vi "Camera Messenger Regular.vi"(0 "Notifier Name":string, 1 "Binning":u16, 2 "General Camera Actions":T3, 5 "Exposure Time (s)":dbl, 7 "Save Path":path, 9 "No. of Frames":u32, 11 "Camera ROI":T1, 12 "Cooler On?":bool, 13 "Defect Correction On?":bool, 14 "Fan On?":bool) -> (3 "Current Exposure Time (s)":dbl, 4 "Notifier Name Dup":string, 6 "Running?":bool, 8 "Camera ROI":T1, 10 "Current Frame":u32, 15 "Image Ref":T2)   [LabVIEW 2016]
uses:
  Camera Controls/Generic Camera Actions.ctl
  Camera Controls/Generic Camera ROI.ctl
  <vilib>/vision/Image Controls.llb/IMAQ Image.ctl
  Hardware Configuration/Hardware Configuration Controls/Company.ctl
  Hamamatsu/Orca Flash/Orca Flash Controls/Orca Flash ROI.ctl
  Hamamatsu/Orca Flash/Orca Flash Controls/Orca Flash Parameters.ctl
  Hamamatsu/Orca Flash/Orca Flash Controls/Orca Flash Parameter List.ctl
  Hamamatsu/Orca Flash/Orca Flash Controls/Orca Flash Actions.ctl
  IDS/IDS Controls/IDS ROI.ctl
  IDS/IDS Controls/IDS Parameters.ctl
  IDS/IDS Controls/IDS Parameter List.ctl
  IDS/IDS Controls/IDS Actions.ctl
  Photometrics/Prime BSI/R Cubed SITK/Prime BSI R3 Controls/Prime R3 ROI.ctl
  Photometrics/Prime BSI/R Cubed SITK/Prime BSI R3 Controls/Prime R3 Parameters.ctl
  Photometrics/Prime BSI/R Cubed SITK/Prime BSI R3 Controls/Prime R3 Parameter List.ctl
  Photometrics/Prime BSI/R Cubed SITK/Prime BSI R3 Controls/Prime R3 Actions.ctl
  Camera Controls/Camera IMAQ Key Info.ctl
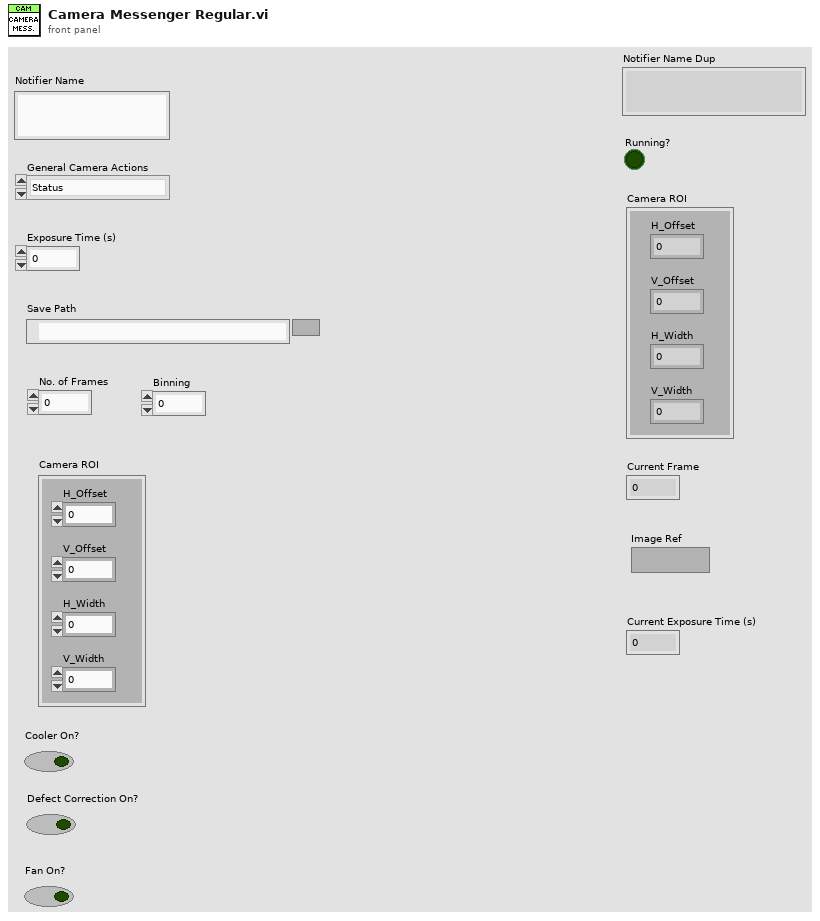
[diagram p1: front panel]
types:
  T1 = typedef "Generic Camera ROI.ctl" = cluster{"H_Offset":u16, "V_Offset":u16, "H_Width":u16, "V_Width":u16}
  T2 = typedef "IMAQ Image.ctl" = refnum<image>
  T3 = typedef "Generic Camera Actions.ctl" = enum16{"Status", "Live Preview", "Capture", "Abort", "Set Exposure Time (s)", "Get Exposure Time (s)", "Record Settings", "Binning", "Set ROI", "Get ROI", "Defect Correction On?", "Cooler On?", "Fan On?", "Quit"}
  T4 = typedef "Company.ctl" = enum16{"AA Opto Electronic", "ASI", "Coherent", "CVI", "DAQmx", "Hamamatsu", "IDS", "Mad City Labs", "Marzhauser", "Measurement Computing", "MPB Com", "Photometrics", "PI", "Prior", "Thorlabs"}
  T5 = typedef "Orca Flash Parameters.ctl" = cluster{"Value":dbl, "Parameter":T6}
  T6 = typedef "Orca Flash Parameter List.ctl" = u32
  T7 = typedef "Orca Flash ROI.ctl" = cluster{"H Offset":i32, "V Offset":i32, "H Width":i32, "V Width":i32}
  T8 = typedef "Orca Flash Actions.ctl" = enum16{"IDLE", "PREVIEW", "RECORD", "Record Settings", "SETPARAM", "GETPARAM", "SETROI", "GETROI", "PROGRESSIVE MODE", "AREA MODE", "STATUS", "QUIT"}
  T9 = typedef "IDS Parameter List.ctl" = enum16{"Exposure Time (s)", "Binning"}
  T10 = typedef "IDS Parameters.ctl" = cluster{"Parameter":T9, "Value":dbl}
  T11 = typedef "IDS ROI.ctl" = cluster{"H Offset":i32, "V Offset":i32, "H Width":i32, "V Width":i32}
  T12 = typedef "IDS Actions.ctl" = enum16{"Error Check", "Initialize", "Preview", "Record", "Abort", "Record Settings", "Set Parameter", "Get Parameter", "Set ROI", "Get ROI", "Status", "Quit"}
  T13 = typedef "Prime R3 Parameter List.ctl" = enum16{"Exposure Time (s)"}
  T14 = typedef "Prime R3 Parameters.ctl" = cluster{"Parameter":T13, "Value":dbl}
  T15 = typedef "Prime R3 ROI.ctl" = cluster{"X Start":u32, "X End":u32, "X Bin":u32, "Y Start":u32, "Y End":u32, "Y Bin":u32}
  T16 = typedef "Prime R3 Actions.ctl" = enum16{"Error Check", "Initialize", "Preview", "Record", "Abort", "Record Settings", "Set Parameter", "Get Parameter", "Set ROI", "Get ROI", "Status", "Set Trigger", "Quit"}
  T17 = typedef "Camera IMAQ Key Info.ctl" = cluster{"Frame":u32, "Sensor Height":i32, "Sensor Width":i32, "ROI Height":i32, "ROI Width":i32, "ROI Enable?":bool, "Bit per Pixel":u8}
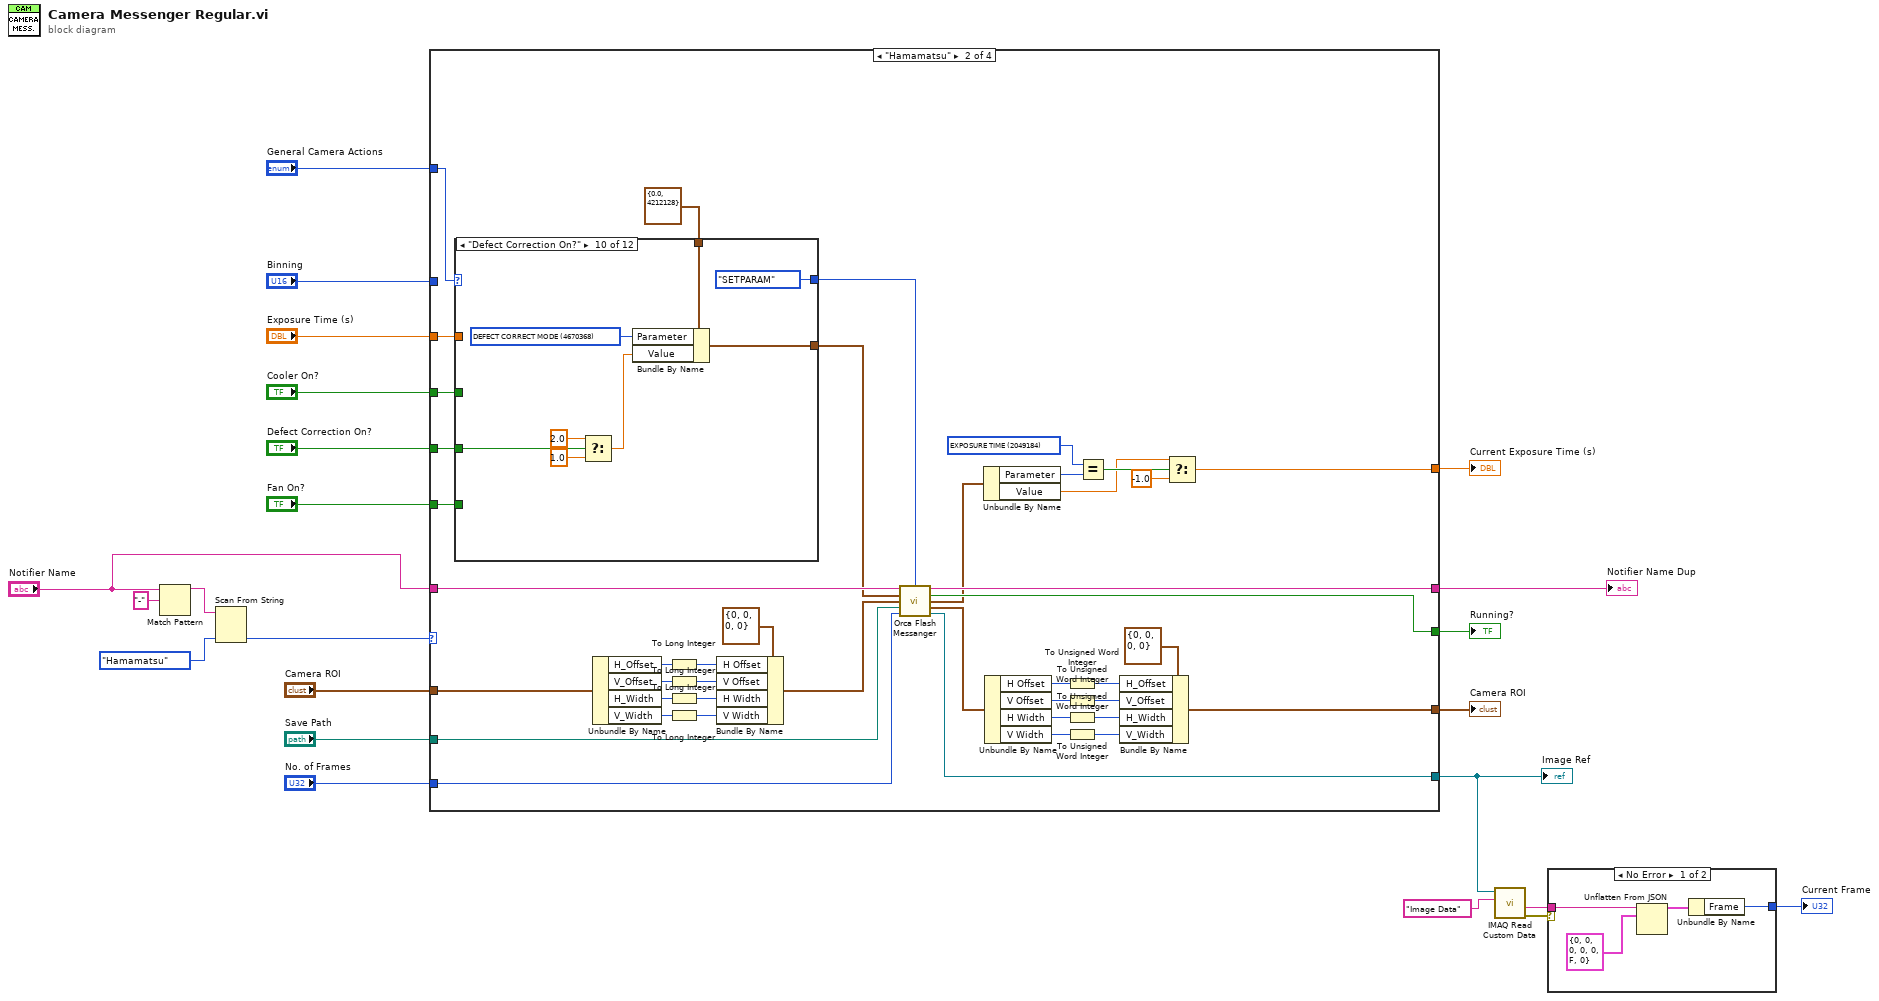
[diagram p0: block diagram]
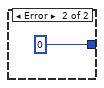
[diagram p2: hidden frame]
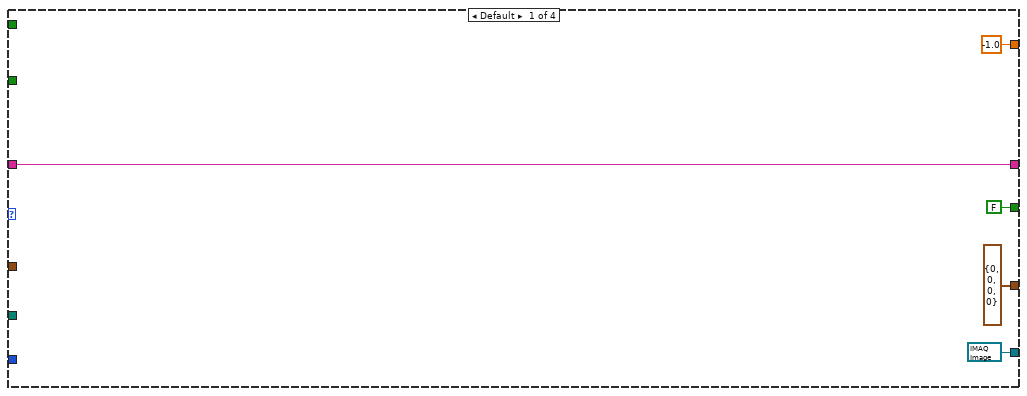
[diagram p3: hidden frame]
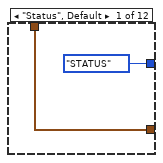
[diagram p4: hidden frame]
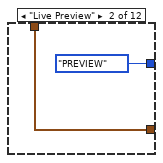
[diagram p5: hidden frame]
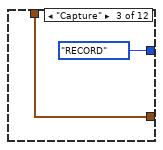
[diagram p6: hidden frame]
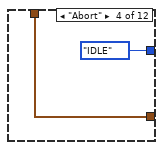
[diagram p7: hidden frame]
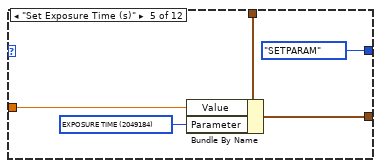
[diagram p8: hidden frame]
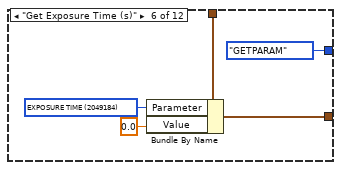
[diagram p9: hidden frame]
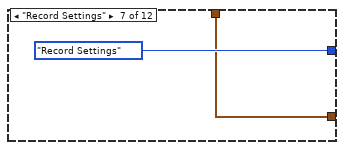
[diagram p10: hidden frame]
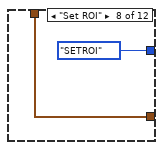
[diagram p11: hidden frame]
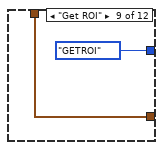
[diagram p12: hidden frame]
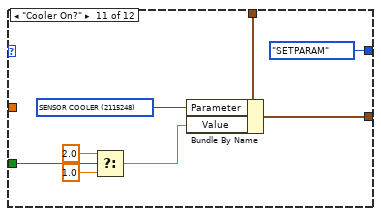
[diagram p13: hidden frame]
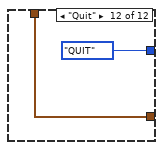
[diagram p14: hidden frame]
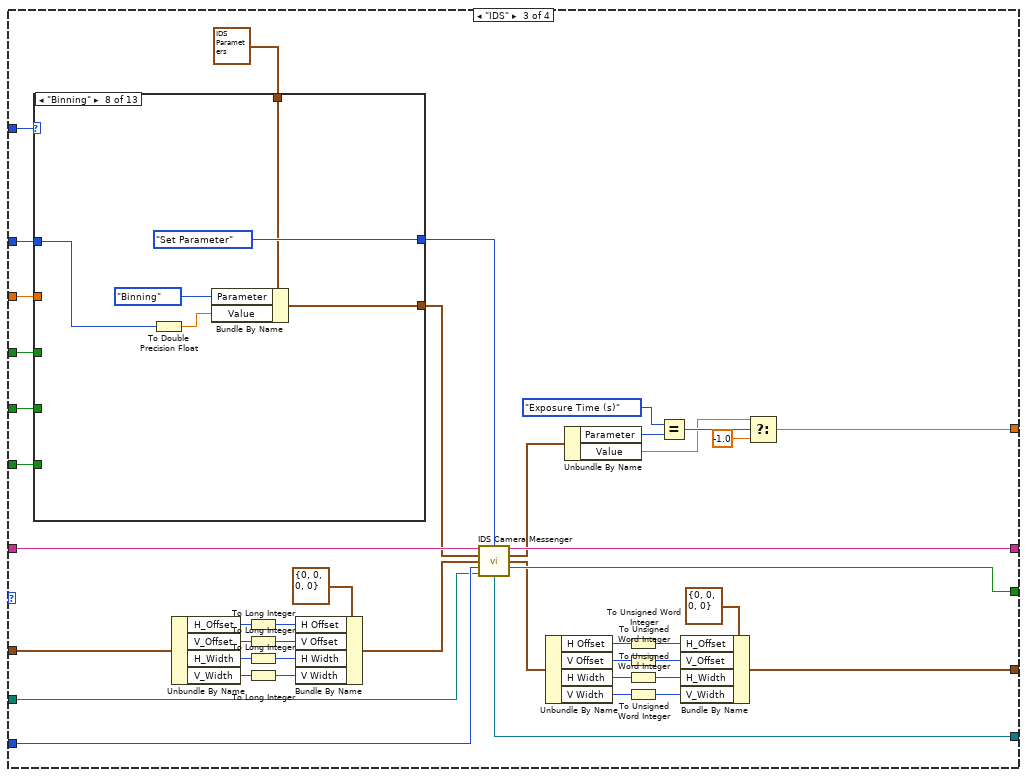
[diagram p15: hidden frame]
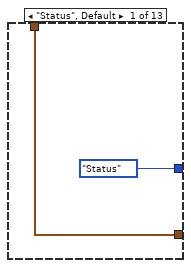
[diagram p16: hidden frame]
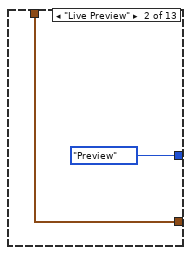
[diagram p17: hidden frame]
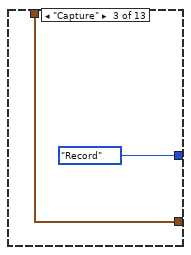
[diagram p18: hidden frame]
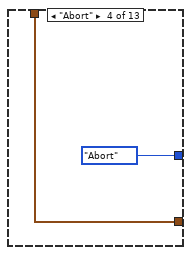
[diagram p19: hidden frame]
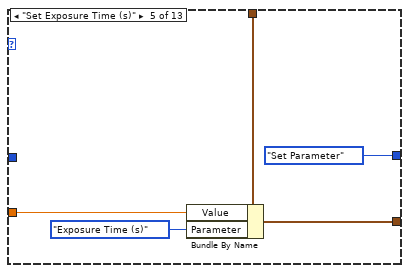
[diagram p20: hidden frame]
diagram:
  n1 = Match Pattern(string="Notifier Name", regular expression="-") -> (before substring=w20:string)  [unwired: 1 in, 3 out]
  n2 = Scan From String(input string=w20, default 1=Company."Hamamatsu" ("Company")) -> (output 1=w21:T4)  [unwired: 3 in, 3 out]
  n3 = case shown="\"Hamamatsu\"" w21 {
    tunnel: "Notifier Name" -> [w28 w71 w157 w239]
    tunnel: "General Camera Actions" -> [_ w56 w142 w232]
    tunnel: "No. of Frames" -> [_ w70 w156 w238]
    tunnel: "Save Path" -> [_ w69 w155 w210]
    tunnel: "Camera ROI" -> [_ w67 w153 w236]
    tunnel: [w28 w57 w143 w233] -> w15
    tunnel: "Exposure Time (s)" -> [_ w51 w138 w228]
    tunnel: "Cooler On?" -> [_ w55 w141 w231]
    tunnel: "Defect Correction On?" -> [_ w54 w140 w230]
    tunnel: "Fan On?" -> [_ w53 w139 w229]
    tunnel: [T2 refnum ("Image Ref") w48 w135 w225] -> w6
    tunnel: [FALSE ("Running?") w47 w134 w224] -> w10
    tunnel: [T1 {"H_Offset"=0, "V_Offset"=0, "H_Width"=0, "V_Width"=0} ("General Camera ROI") w36 w123 w213] -> w9
    tunnel: [-1.0 ("f") w30 w115 w195] -> w2
    tunnel: "Binning" -> [_ _ w114 _]
    frame Default {
    }
    frame "Hamamatsu" {
      w29 = T6 2049184 items=["SENSOR MODE"=4212128, "READOUT SPEED"=4211872, "READOUT DIRECTION"=4211904, "TRIGGER GLOBAL EXPOSURE"=2049680, "TRIGGER DELAY"=1066480, "SYNC READOUT SYSTEM BLANK"=1066528, "SENSOR COOLER"=2115248, "SENSOR COOLER STATUS"=2115280, "EXPOSURE TIME"=2049184, "DEFECT CORRECT MODE"=4670368, "BINNING"=4215968, "INTERNAL LINE SPEED"=4226000, "INTERNAL LINE INTERVAL"=4226016, "IMAGE PIXEL TYPE"=4343296, "NUMBER OF OUTPUT TRIGGER CONNECTOR"=1852320, "OUTPUT TRIGGER SOURCE[0]"=1852576, "OUTPUT TRIGGER SOURCE[1]"=1852832, "OUTPUT TRIGGER SOURCE[2]"=1853088, "OUTPUT TRIGGER POLARITY[0]"=1852592, "OUTPUT TRIGGER POLARITY[1]"=1852848, "OUTPUT TRIGGER POLARITY[2]"=1853104, "OUTPUT TRIGGER ACTIVE[0]"=1852608, "OUTPUT TRIGGER ACTIVE[1]"=1852864, "OUTPUT TRIGGER ACTIVE[2]"=1853120, "OUTPUT TRIGGER DELAY[0]"=1852624, "OUTPUT TRIGGER DELAY[1]"=1852880, "OUTPUT TRIGGER DELAY[2]"=1853136, "OUTPUT TRIGGER PERIOD[0]"=1852640, "OUTPUT TRIGGER PERIOD[1]"=1852896, "OUTPUT TRIGGER PERIOD[2]"=1853152, "OUTPUT TRIGGER KIND[0]"=1852656, "OUTPUT TRIGGER KIND[1]"=1852912, "OUTPUT TRIGGER KIND[2]"=1853168, "OUTPUT TRIGGER PRE HSYNC COUNT"=1852704] ("x")
      n4 = case shown="\"Defect Correction On?\"" w56 {
        tunnel: w55 -> [_ _ _ _ _ _ _ _ _ _ w108 _]
        tunnel: w54 -> [_ _ _ _ _ _ _ _ _ w99 _ _]
        tunnel: w53 -> [_ _ _ _ _ _ _ _ _ _ _ _]
        tunnel: [Orca_Flash_Actions."STATUS" ("Camera Actions") Orca_Flash_Actions."PREVIEW" ("Camera Actions") Orca_Flash_Actions."RECORD" ("Camera Actions") Orca_Flash_Actions."IDLE" ("Camera Actions") Orca_Flash_Actions."SETPARAM" ("Camera Actions") Orca_Flash_Actions."GETPARAM" ("Camera Actions") Orca_Flash_Actions."Record Settings" ("Camera Actions") Orca_Flash_Actions."SETROI" ("Camera Actions") Orca_Flash_Actions."GETROI" ("Camera Actions") Orca_Flash_Actions."SETPARAM" ("Camera Actions") Orca_Flash_Actions."SETPARAM" ("Camera Actions") Orca_Flash_Actions."QUIT" ("Camera Actions")] -> w52
        tunnel: w51 -> [_ _ _ _ w83 _ _ _ _ _ _ _]
        tunnel: [w72 w74 w76 w78 w82 w88 w90 w92 w94 w101 w104 w113] -> w50
        tunnel: T5 {"Value"=0.0, "Parameter"=4212128} ("sCMOS Parameter") -> [w72 w74 w76 w78 w81 w89 w90 w92 w94 w102 w110 w113]
        frame "Status", Default {
        }
        frame "Live Preview" {
        }
        frame "Capture" {
        }
        frame "Abort" {
        }
        frame "Set Exposure Time (s)" {
          w80 = T6 2049184 items=["SENSOR MODE"=4212128, "READOUT SPEED"=4211872, "READOUT DIRECTION"=4211904, "TRIGGER GLOBAL EXPOSURE"=2049680, "TRIGGER DELAY"=1066480, "SYNC READOUT SYSTEM BLANK"=1066528, "SENSOR COOLER"=2115248, "SENSOR COOLER STATUS"=2115280, "EXPOSURE TIME"=2049184, "DEFECT CORRECT MODE"=4670368, "BINNING"=4215968, "INTERNAL LINE SPEED"=4226000, "INTERNAL LINE INTERVAL"=4226016, "IMAGE PIXEL TYPE"=4343296, "NUMBER OF OUTPUT TRIGGER CONNECTOR"=1852320, "OUTPUT TRIGGER SOURCE[0]"=1852576, "OUTPUT TRIGGER SOURCE[1]"=1852832, "OUTPUT TRIGGER SOURCE[2]"=1853088, "OUTPUT TRIGGER POLARITY[0]"=1852592, "OUTPUT TRIGGER POLARITY[1]"=1852848, "OUTPUT TRIGGER POLARITY[2]"=1853104, "OUTPUT TRIGGER ACTIVE[0]"=1852608, "OUTPUT TRIGGER ACTIVE[1]"=1852864, "OUTPUT TRIGGER ACTIVE[2]"=1853120, "OUTPUT TRIGGER DELAY[0]"=1852624, "OUTPUT TRIGGER DELAY[1]"=1852880, "OUTPUT TRIGGER DELAY[2]"=1853136, "OUTPUT TRIGGER PERIOD[0]"=1852640, "OUTPUT TRIGGER PERIOD[1]"=1852896, "OUTPUT TRIGGER PERIOD[2]"=1853152, "OUTPUT TRIGGER KIND[0]"=1852656, "OUTPUT TRIGGER KIND[1]"=1852912, "OUTPUT TRIGGER KIND[2]"=1853168, "OUTPUT TRIGGER PRE HSYNC COUNT"=1852704] ("Parameter")
          n5 = Bundle By Name(cluster=w81, "Value"=w83, "Parameter"=w80) -> (w82:T5)
        }
        frame "Get Exposure Time (s)" {
          w86 = T6 2049184 items=["SENSOR MODE"=4212128, "READOUT SPEED"=4211872, "READOUT DIRECTION"=4211904, "TRIGGER GLOBAL EXPOSURE"=2049680, "TRIGGER DELAY"=1066480, "SYNC READOUT SYSTEM BLANK"=1066528, "SENSOR COOLER"=2115248, "SENSOR COOLER STATUS"=2115280, "EXPOSURE TIME"=2049184, "DEFECT CORRECT MODE"=4670368, "BINNING"=4215968, "INTERNAL LINE SPEED"=4226000, "INTERNAL LINE INTERVAL"=4226016, "IMAGE PIXEL TYPE"=4343296, "NUMBER OF OUTPUT TRIGGER CONNECTOR"=1852320, "OUTPUT TRIGGER SOURCE[0]"=1852576, "OUTPUT TRIGGER SOURCE[1]"=1852832, "OUTPUT TRIGGER SOURCE[2]"=1853088, "OUTPUT TRIGGER POLARITY[0]"=1852592, "OUTPUT TRIGGER POLARITY[1]"=1852848, "OUTPUT TRIGGER POLARITY[2]"=1853104, "OUTPUT TRIGGER ACTIVE[0]"=1852608, "OUTPUT TRIGGER ACTIVE[1]"=1852864, "OUTPUT TRIGGER ACTIVE[2]"=1853120, "OUTPUT TRIGGER DELAY[0]"=1852624, "OUTPUT TRIGGER DELAY[1]"=1852880, "OUTPUT TRIGGER DELAY[2]"=1853136, "OUTPUT TRIGGER PERIOD[0]"=1852640, "OUTPUT TRIGGER PERIOD[1]"=1852896, "OUTPUT TRIGGER PERIOD[2]"=1853152, "OUTPUT TRIGGER KIND[0]"=1852656, "OUTPUT TRIGGER KIND[1]"=1852912, "OUTPUT TRIGGER KIND[2]"=1853168, "OUTPUT TRIGGER PRE HSYNC COUNT"=1852704] ("Parameter")
          n6 = Bundle By Name(cluster=w89, "Parameter"=w86, "Value"=0.0) -> (w88:T5)
        }
        frame "Record Settings" {
        }
        frame "Set ROI" {
        }
        frame "Get ROI" {
        }
        frame "Defect Correction On?" {
          w100 = T6 4670368 items=["SENSOR MODE"=4212128, "READOUT SPEED"=4211872, "READOUT DIRECTION"=4211904, "TRIGGER GLOBAL EXPOSURE"=2049680, "TRIGGER DELAY"=1066480, "SYNC READOUT SYSTEM BLANK"=1066528, "SENSOR COOLER"=2115248, "SENSOR COOLER STATUS"=2115280, "EXPOSURE TIME"=2049184, "DEFECT CORRECT MODE"=4670368, "BINNING"=4215968, "INTERNAL LINE SPEED"=4226000, "INTERNAL LINE INTERVAL"=4226016, "IMAGE PIXEL TYPE"=4343296, "NUMBER OF OUTPUT TRIGGER CONNECTOR"=1852320, "OUTPUT TRIGGER SOURCE[0]"=1852576, "OUTPUT TRIGGER SOURCE[1]"=1852832, "OUTPUT TRIGGER SOURCE[2]"=1853088, "OUTPUT TRIGGER POLARITY[0]"=1852592, "OUTPUT TRIGGER POLARITY[1]"=1852848, "OUTPUT TRIGGER POLARITY[2]"=1853104, "OUTPUT TRIGGER ACTIVE[0]"=1852608, "OUTPUT TRIGGER ACTIVE[1]"=1852864, "OUTPUT TRIGGER ACTIVE[2]"=1853120, "OUTPUT TRIGGER DELAY[0]"=1852624, "OUTPUT TRIGGER DELAY[1]"=1852880, "OUTPUT TRIGGER DELAY[2]"=1853136, "OUTPUT TRIGGER PERIOD[0]"=1852640, "OUTPUT TRIGGER PERIOD[1]"=1852896, "OUTPUT TRIGGER PERIOD[2]"=1853152, "OUTPUT TRIGGER KIND[0]"=1852656, "OUTPUT TRIGGER KIND[1]"=1852912, "OUTPUT TRIGGER KIND[2]"=1853168, "OUTPUT TRIGGER PRE HSYNC COUNT"=1852704] ("Parameter")
          n7 = Select(t=2.0, s=w99, f=1.0) -> (s? t:f=w96:dbl)
          n8 = Bundle By Name(cluster=w102, "Parameter"=w100, "Value"=w96) -> (w101:T5)
        }
        frame "Cooler On?" {
          w109 = T6 2115248 items=["SENSOR MODE"=4212128, "READOUT SPEED"=4211872, "READOUT DIRECTION"=4211904, "TRIGGER GLOBAL EXPOSURE"=2049680, "TRIGGER DELAY"=1066480, "SYNC READOUT SYSTEM BLANK"=1066528, "SENSOR COOLER"=2115248, "SENSOR COOLER STATUS"=2115280, "EXPOSURE TIME"=2049184, "DEFECT CORRECT MODE"=4670368, "BINNING"=4215968, "INTERNAL LINE SPEED"=4226000, "INTERNAL LINE INTERVAL"=4226016, "IMAGE PIXEL TYPE"=4343296, "NUMBER OF OUTPUT TRIGGER CONNECTOR"=1852320, "OUTPUT TRIGGER SOURCE[0]"=1852576, "OUTPUT TRIGGER SOURCE[1]"=1852832, "OUTPUT TRIGGER SOURCE[2]"=1853088, "OUTPUT TRIGGER POLARITY[0]"=1852592, "OUTPUT TRIGGER POLARITY[1]"=1852848, "OUTPUT TRIGGER POLARITY[2]"=1853104, "OUTPUT TRIGGER ACTIVE[0]"=1852608, "OUTPUT TRIGGER ACTIVE[1]"=1852864, "OUTPUT TRIGGER ACTIVE[2]"=1853120, "OUTPUT TRIGGER DELAY[0]"=1852624, "OUTPUT TRIGGER DELAY[1]"=1852880, "OUTPUT TRIGGER DELAY[2]"=1853136, "OUTPUT TRIGGER PERIOD[0]"=1852640, "OUTPUT TRIGGER PERIOD[1]"=1852896, "OUTPUT TRIGGER PERIOD[2]"=1853152, "OUTPUT TRIGGER KIND[0]"=1852656, "OUTPUT TRIGGER KIND[1]"=1852912, "OUTPUT TRIGGER KIND[2]"=1853168, "OUTPUT TRIGGER PRE HSYNC COUNT"=1852704] ("Parameter")
          n9 = Select(t=2.0, s=w108, f=1.0) -> (s? t:f=w105:dbl)
          n10 = Bundle By Name(cluster=w110, "Parameter"=w109, "Value"=w105) -> (w104:T5)
        }
        frame "Quit" {
        }
      }
      n11 = Unbundle By Name(w67) -> ("H_Offset"=w63:u16, "V_Offset"=w64:u16, "H_Width"=w65:u16, "V_Width"=w66:u16)
      n12 = To Long Integer(number=w63) -> (32bit integer=w62:i32)
      n13 = To Long Integer(number=w64) -> (32bit integer=w61:i32)
      n14 = To Long Integer(number=w65) -> (32bit integer=w60:i32)
      n15 = To Long Integer(number=w66) -> (32bit integer=w59:i32)
      n16 = Bundle By Name(cluster=T7 {"H Offset"=0, "V Offset"=0, "H Width"=0, "V Width"=0} ("sCMOS ROI"), "H Offset"=w62, "V Offset"=w61, "H Width"=w60, "V Width"=w59) -> (w58:T7)
      n17 = call "Orca Flash Messanger.vi"("Notifier Name"=w71, "Camera Actions"=w52, "sCMOS Parameter"=w50, "sCMOS ROI"=w58, "Path"=w69, "# of frames"=w70) -> ("Notifier Name Dup"=w57:string, "Running?"=w47:bool, "sCMOS Parameter"=w31:T5, "sCMOS ROI"=w45:T7, "Image Ref"=w48:T2)  [unwired: 5 in]
      n18 = Unbundle By Name(w31) -> ("Parameter"=w35:T6, "Value"=w33:dbl)
      n19 = Unbundle By Name(w45) -> ("H Offset"=w44:i32, "V Offset"=w43:i32, "H Width"=w42:i32, "V Width"=w41:i32)
      n20 = To Unsigned Word Integer(number=w44) -> (unsigned 16bit integer=w40:u16)
      n21 = To Unsigned Word Integer(number=w43) -> (unsigned 16bit integer=w39:u16)
      n22 = To Unsigned Word Integer(number=w42) -> (unsigned 16bit integer=w38:u16)
      n23 = To Unsigned Word Integer(number=w41) -> (unsigned 16bit integer=w37:u16)
      n24 = Equal?(x=w29, y=w35) -> (x = y?=w34:bool)
      n25 = Bundle By Name(cluster=T1 {"H_Offset"=0, "V_Offset"=0, "H_Width"=0, "V_Width"=0} ("General Camera ROI"), "H_Offset"=w40, "V_Offset"=w39, "H_Width"=w38, "V_Width"=w37) -> (w36:T1)
      n26 = Select(t=w33, s=w34, f=-1.0) -> (s? t:f=w30:dbl)
    }
    frame "IDS" {
      n27 = case shown="\"Binning\"" w142 {
        tunnel: w141 -> [_ _ _ _ _ _ _ _ _ _ _ _ _]
        tunnel: w140 -> [_ _ _ _ _ _ _ _ _ _ _ _ _]
        tunnel: w139 -> [_ _ _ _ _ _ _ _ _ _ _ _ _]
        tunnel: [IDS_Actions."Status" ("IDS Actions") IDS_Actions."Preview" ("IDS Actions") IDS_Actions."Record" ("IDS Actions") IDS_Actions."Abort" ("IDS Actions") IDS_Actions."Set Parameter" ("IDS Actions") IDS_Actions."Get Parameter" ("IDS Actions") IDS_Actions."Record Settings" ("IDS Actions") IDS_Actions."Set Parameter" ("IDS Actions") IDS_Actions."Set ROI" ("IDS Actions") IDS_Actions."Get ROI" ("IDS Actions") IDS_Actions."Status" ("IDS Actions") IDS_Actions."Status" ("IDS Actions") IDS_Actions."Quit" ("IDS Actions")] -> w122
        tunnel: w138 -> [_ _ _ _ w170 _ _ _ _ _ _ _ _]
        tunnel: [w159 w161 w163 w165 w169 w171 w177 w181 w185 w187 w189 w191 w193] -> w137
        tunnel: T10 {"Parameter"=enum."Exposure Time (s)", "Value"=4212128.0} ("IDS Parameter") -> [w159 w161 w163 w165 w168 w174 w177 w182 w185 w187 w189 w191 w193]
        tunnel: w114 -> [_ _ _ _ _ _ _ w178 _ _ _ _ _]
        frame "Status", Default {
        }
        frame "Live Preview" {
        }
        frame "Capture" {
        }
        frame "Abort" {
        }
        frame "Set Exposure Time (s)" {
          n28 = Bundle By Name(cluster=w168, "Value"=w170, "Parameter"=IDS_Parameter_List."Exposure Time (s)") -> (w169:T10)
        }
        frame "Get Exposure Time (s)" {
          n29 = Bundle By Name(cluster=w174, "Parameter"=IDS_Parameter_List."Exposure Time (s)", "Value"=0.0) -> (w171:T10)
        }
        frame "Record Settings" {
        }
        frame "Binning" {
          n30 = To Double Precision Float(number=w178) -> (double precision float=w179:dbl)
          n31 = Bundle By Name(cluster=w182, "Parameter"=IDS_Parameter_List."Binning", "Value"=w179) -> (w181:T10)
        }
        frame "Set ROI" {
        }
        frame "Get ROI" {
        }
        frame "Defect Correction On?" {
        }
        frame "Cooler On?" {
        }
        frame "Quit" {
        }
      }
      n32 = Unbundle By Name(w153) -> ("H_Offset"=w149:u16, "V_Offset"=w150:u16, "H_Width"=w151:u16, "V_Width"=w152:u16)
      n33 = To Long Integer(number=w149) -> (32bit integer=w148:i32)
      n34 = To Long Integer(number=w150) -> (32bit integer=w147:i32)
      n35 = To Long Integer(number=w151) -> (32bit integer=w146:i32)
      n36 = To Long Integer(number=w152) -> (32bit integer=w145:i32)
      n37 = Bundle By Name(cluster=T11 {"H Offset"=0, "V Offset"=0, "H Width"=0, "V Width"=0} ("sCMOS ROI"), "H Offset"=w148, "V Offset"=w147, "H Width"=w146, "V Width"=w145) -> (w144:T11)
      n38 = call "IDS Camera Messenger.vi"("Notifier Name"=w157, "IDS Actions"=w122, "IDS Parameter"=w137, "ROI Setup"=w144, "# of Frames"=w156, "File Save Path"=w155) -> ("Notifier Name (Dup)"=w143:string, "IDS Parameter"=w121:T10, "IDS ROI"=w132:T11, "Running?"=w134:bool, "Image Ref"=w135:T2)  [unwired: 4 in, 1 out]
      n39 = Unbundle By Name(w132) -> ("H Offset"=w131:i32, "V Offset"=w130:i32, "H Width"=w129:i32, "V Width"=w128:i32)
      n40 = Unbundle By Name(w121) -> ("Parameter"=w120:T9, "Value"=w117:dbl)
      n41 = To Unsigned Word Integer(number=w131) -> (unsigned 16bit integer=w127:u16)
      n42 = To Unsigned Word Integer(number=w130) -> (unsigned 16bit integer=w126:u16)
      n43 = To Unsigned Word Integer(number=w129) -> (unsigned 16bit integer=w125:u16)
      n44 = To Unsigned Word Integer(number=w128) -> (unsigned 16bit integer=w124:u16)
      n45 = Equal?(x=IDS_Parameter_List."Exposure Time (s)", y=w120) -> (x = y?=w118:bool)
      n46 = Bundle By Name(cluster=T1 {"H_Offset"=0, "V_Offset"=0, "H_Width"=0, "V_Width"=0} ("General Camera ROI"), "H_Offset"=w127, "V_Offset"=w126, "H_Width"=w125, "V_Width"=w124) -> (w123:T1)
      n47 = Select(t=w117, s=w118, f=-1.0) -> (s? t:f=w115:dbl)
    }
    frame "Photometrics" {
      w211 = u32 1 ("number")
      n48 = case shown="\"Record Settings\"" w232 {
        tunnel: w231 -> [_ _ _ _ _ _ _ _ _ _ _ _]
        tunnel: w230 -> [_ _ _ _ _ _ _ _ _ _ _ _]
        tunnel: w229 -> [_ _ _ _ _ _ _ _ _ _ _ _]
        tunnel: [Prime_R3_Actions."Status" ("Prime Actions") Prime_R3_Actions."Preview" ("Prime Actions") Prime_R3_Actions."Record" ("Prime Actions") Prime_R3_Actions."Abort" ("Prime Actions") Prime_R3_Actions."Set Parameter" ("Prime Actions") Prime_R3_Actions."Get Parameter" ("Prime Actions") Prime_R3_Actions."Record Settings" ("Prime Actions") Prime_R3_Actions."Set ROI" ("Prime Actions") Prime_R3_Actions."Get ROI" ("Prime Actions") Prime_R3_Actions."Status" ("Prime Actions") Prime_R3_Actions."Status" ("Prime Actions") Prime_R3_Actions."Quit" ("Prime Actions")] -> w212
        tunnel: w228 -> [_ _ _ _ w252 _ _ _ _ _ _ _]
        tunnel: [w241 w243 w245 w247 w251 w255 w259 w261 w263 w265 w267 w269] -> w227
        tunnel: T14 {"Parameter"=enum."Exposure Time (s)", "Value"=4212128.0} ("Prime Parameter") -> [w241 w243 w245 w247 w250 w256 w259 w261 w263 w265 w267 w269]
        frame "Status", Default {
        }
        frame "Live Preview" {
        }
        frame "Capture" {
        }
        frame "Abort" {
        }
        frame "Set Exposure Time (s)" {
          n49 = Bundle By Name(cluster=w250, "Value"=w252, "Parameter"=Prime_R3_Parameter_List."Exposure Time (s)") -> (w251:T14)
        }
        frame "Get Exposure Time (s)" {
          n50 = Bundle By Name(cluster=w256, "Parameter"=Prime_R3_Parameter_List."Exposure Time (s)", "Value"=0.0) -> (w255:T14)
        }
        frame "Record Settings" {
        }
        frame "Set ROI" {
        }
        frame "Get ROI" {
        }
        frame "Defect Correction On?" {
        }
        frame "Cooler On?" {
        }
        frame "Quit" {
        }
      }
      n51 = Unbundle By Name(w236) -> ("V_Offset"=w202:u16, "V_Width"=w204:u16, "H_Offset"=w208:u16, "H_Width"=w209:u16)
      n52 = Add(x=w202, y=w204) -> (x+y=w203:u16)
      n53 = Add(x=w208, y=w209) -> (x+y=w206:u16)
      n54 = To Unsigned Long Integer(number=w202) -> (unsigned 32bit integer=w201:u32)
      n55 = To Unsigned Long Integer(number=w203) -> (unsigned 32bit integer=w235:u32)
      n56 = To Unsigned Long Integer(number=w208) -> (unsigned 32bit integer=w207:u32)
      n57 = To Unsigned Long Integer(number=w206) -> (unsigned 32bit integer=w205:u32)
      n58 = Bundle By Name(cluster=T15 {"X Start"=0, "X End"=0, "X Bin"=0, "Y Start"=0, "Y End"=0, "Y Bin"=0} ("sCMOS ROI"), "X Start"=w201, "X End"=w235, "X Bin"=w211, "Y Start"=w207, "Y End"=w205, "Y Bin"=w211) -> (w234:T15)
      n59 = call "Prime BSI R3 Camera Messenger.vi"("Notifier Name"=w239, "Prime Actions"=w212, "Prime Parameter"=w227, "ROI Setup"=w234, "# of Frames"=w238, "File Save Path"=w210) -> ("Notifier Name (Dup)"=w233:string, "Prime Parameter"=w196:T14, "Prime ROI"=w222:T15, "Running?"=w224:bool, "Image Ref"=w225:T2)  [unwired: 4 in, 1 out]
      n60 = Unbundle By Name(w222) -> ("X Start"=w221:u32, "X End"=w220:u32, "X Bin"=w219:u32, "Y Start"=w218:u32)
      n61 = Unbundle By Name(w196) -> ("Parameter"=w200:T13, "Value"=w198:dbl)
      n62 = To Unsigned Word Integer(number=w221) -> (unsigned 16bit integer=w217:u16)
      n63 = To Unsigned Word Integer(number=w220) -> (unsigned 16bit integer=w216:u16)
      n64 = To Unsigned Word Integer(number=w219) -> (unsigned 16bit integer=w215:u16)
      n65 = To Unsigned Word Integer(number=w218) -> (unsigned 16bit integer=w214:u16)
      n66 = Bundle By Name(cluster=T1 {"H_Offset"=0, "V_Offset"=0, "H_Width"=0, "V_Width"=0} ("General Camera ROI"), "H_Offset"=w217, "V_Offset"=w216, "H_Width"=w215, "V_Width"=w214) -> (w213:T1)
      n67 = Equal?(x=Prime_R3_Parameter_List."Exposure Time (s)", y=w200) -> (x = y?=w199:bool)
      n68 = Select(t=w198, s=w199, f=-1.0) -> (s? t:f=w195:dbl)
    }
  }
  "Notifier Name Dup" <- w15
  "Image Ref" <- w6
  "Running?" <- w10
  "Camera ROI" <- w9
  "Current Exposure Time (s)" <- w2
  n69 = call "IMAQ Read Custom Data"("Key"="Image Data", "Image"=w6) -> ("error out"=w5:errorcluster, "Custom Data Out"=w7:string)  [unwired: 7 in, 1 out]
  n70 = case shown="No Error" w5 {
    tunnel: w7 -> [w273 _]
    tunnel: [w270 u32 0 ("Frame")] -> w4
    frame No Error {
      n71 = Unflatten From JSON(JSON string=w273, type and defaults=T17 {"Frame"=0, "Sensor Height"=0, "Sensor Width"=0, "ROI Height"=0, "ROI Width"=0, "ROI Enable?"=FALSE, "Bit per Pixel"=0} ("Camera IMAQ Key Info")) -> (value=w271:T17)  [unwired: 5 in, 1 out]
      n72 = Unbundle By Name(w271) -> ("Frame"=w270:u32)
    }
    frame Error {
    }
  }
  "Current Frame" <- w4
